vi "Test U8 Comm.vi"() -> ()   [LabVIEW 2021]
uses:
  ChannelCommon/typedef/Direction.ctl
  ChannelCommon/typedef/TimeStamps.ctl
  CIF_Iceoryx_PCAP_Universal.lvclass
  Iceorxy Utilities/Typedef/PCAP Config.ctl
  ChannelCommon/typedef/New FIFO Config.ctl
  ChannelCommon/typedef/FIFO Flags.ctl
  Iceorxy Utilities/Typedef/PCAP Linktype.ctl
  ChannelCommon/ChannelCommon.lvlib
  Iceorxy Utilities/Iceoryx Channel Utilities.lvlib
panel:
  out "status":string
  out "pass":bool
  out "error out":errorcluster
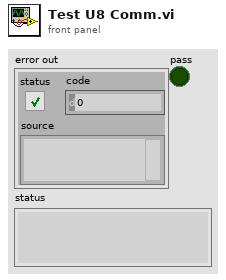
[diagram p1: front panel]
types:
  T1 = typedef "ChannelCommon.lvlib/Direction.ctl" = enum8{"Publisher", "Subscriber"}
  T2 = typedef "Iceoryx Channel Utilities.lvlib/PCAP Config.ctl" = cluster{"New FIFO Config":T3, "Linktype":T5, "Linktype Override":u32, "Type Name Override":string}
  T3 = typedef "ChannelCommon.lvlib/New FIFO Config.ctl" = cluster{"Max Bytes/Msg":u64, "Max Msg/FIFO":u64, "FIFO Flags":T4, "Best Effort Subscribers":u32, "Backpressure Subscribers":u32}
  T4 = typedef "ChannelCommon.lvlib/FIFO Flags.ctl" = cluster{"Backpressure":bool, "Extended Config":bool}
  T5 = typedef "Iceoryx Channel Utilities.lvlib/PCAP Linktype.ctl" = u32
  T6 = typedef "ChannelCommon.lvlib/TimeStamps.ctl" = cluster{"ClockID":u8, "T0":i64, "T_Out":i64}
  T7 = typedef "ChannelCommon.lvlib/New FIFO Instance Response.ctl" = cluster{"Publisher":string, "Custom Data":u8[]}
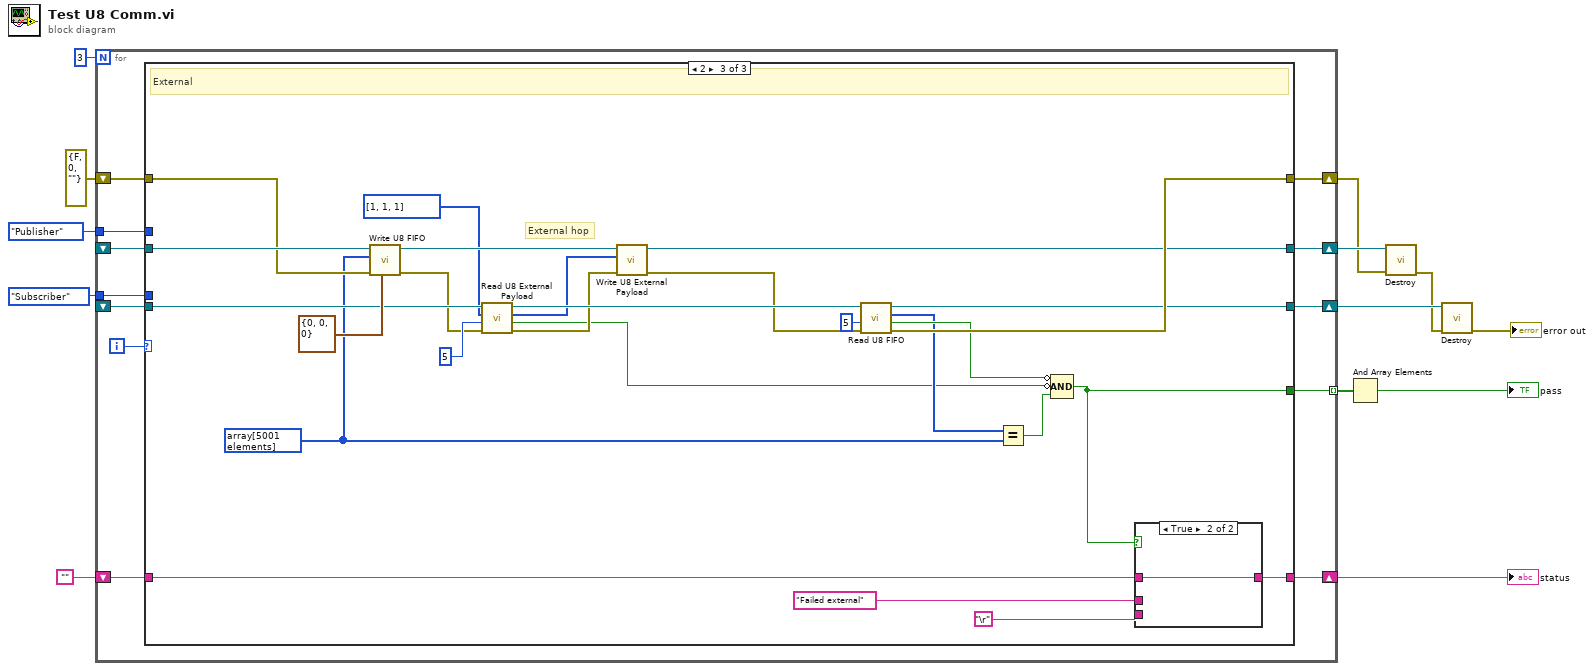
[diagram p0: block diagram]
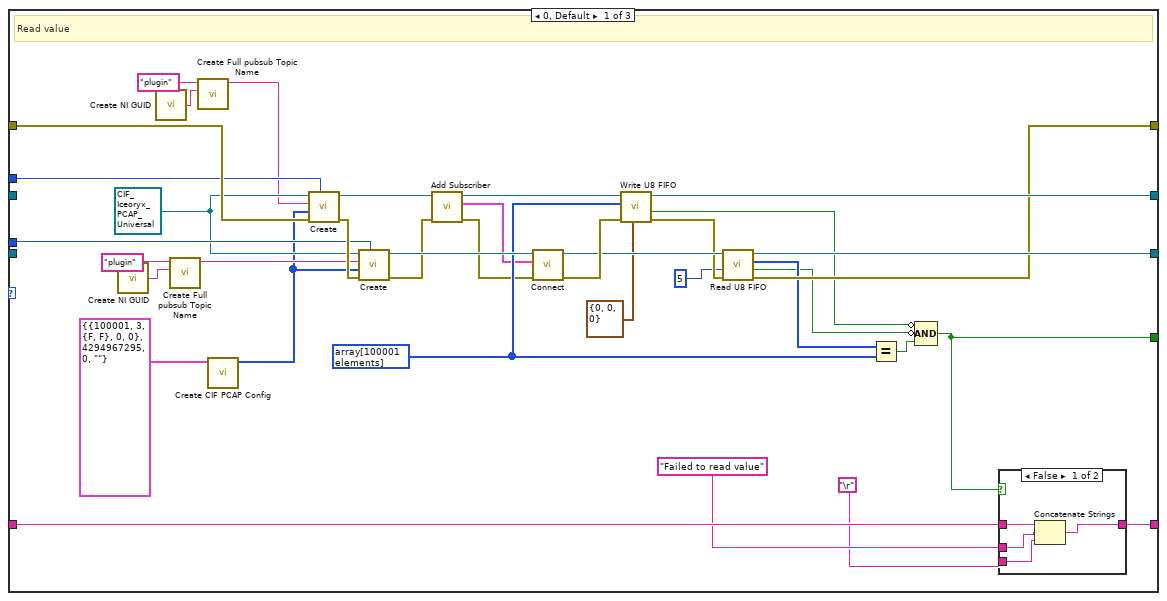
[diagram p2: hidden frame]
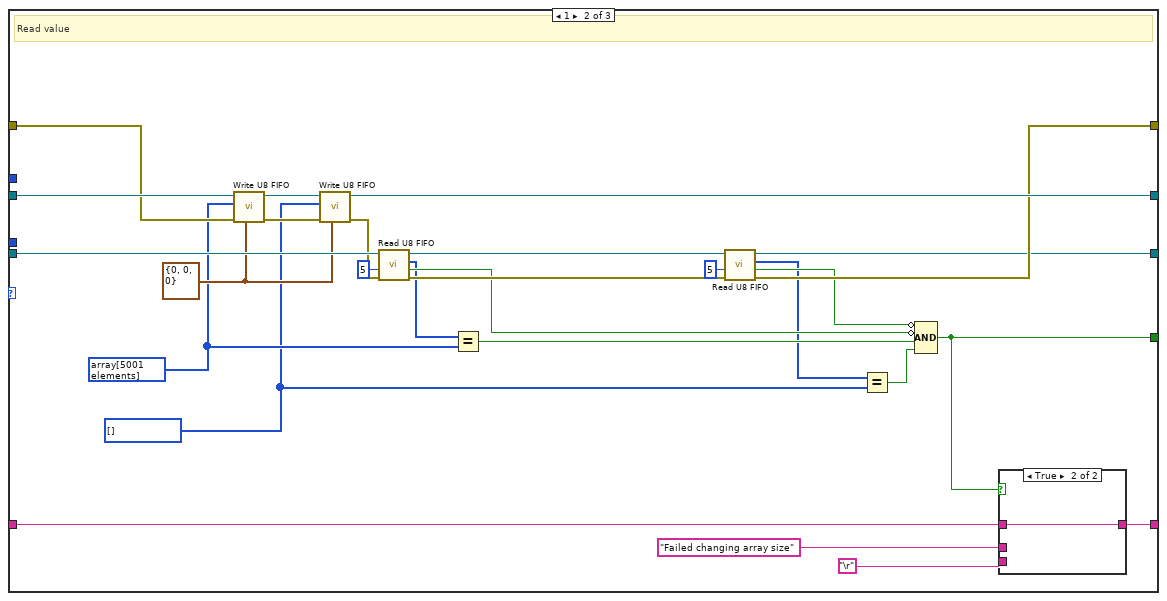
[diagram p4: hidden frame]
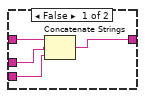
[diagram p5: hidden frame]
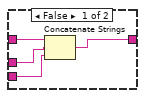
[diagram p6: hidden frame]
diagram:
  n1 = for {
    N: 3 -> [_]
    tunnel: [w25] -> w13 mode=indexing
    shift-right: [w23] -> w3
    shift-left: errorcluster {"status"=FALSE, "code"=0, "source"=""} ("error out") -> [w24]
    shift-right: [w20] -> w9
    shift-left: "" -> [w21]
    tunnel: Direction."Subscriber" ("Direction") -> [w19]
    tunnel: Direction."Publisher" ("Direction") -> [w18]
    shift-right: [w17] -> w5
    shift-left: _ -> [w15]
    shift-right: [w16] -> w4
    shift-left: _ -> [w14]
    i -> [w22]
    n2 = case shown="2" w22 {
      tunnel: [w57 w90 w121] -> w25
      tunnel: w24 -> [w55 w86 w118]
      tunnel: [w47 w79 w117] -> w23
      tunnel: w21 -> [w62 w94 w125]
      tunnel: [w61 w93 w124] -> w20
      tunnel: w19 -> [w54 _ _]
      tunnel: w18 -> [w53 _ _]
      tunnel: [w48 w76 w115] -> w17
      tunnel: [w50 w83 w103] -> w16
      tunnel: w14 -> [_ w87 w119]
      tunnel: w15 -> [_ w82 w111]
      frame 0, Default {
        w40 = refnum<class "CIF_Iceoryx_PCAP_Universal.lvclass"> refnum ("CIF_CIPC_Fifo_U8.lvclass")
        w41 = u8[] array[100001 elements] ("U8 Data")
        # "Read value"
        n3 = call <vilib>:"Create NI GUID.vi"() -> ("NI GUID"=w29:string)
        n4 = call <vilib>:"Create NI GUID.vi"() -> ("NI GUID"=w32:string)
        n5 = call "Create Full pubsub Topic Name.vi"("Topic"=w29, "Plugin name"="plugin") -> ("Full Topic"=w28:string)  [unwired: 8 in, 1 out]
        n6 = call "Create Full pubsub Topic Name.vi"("Topic"=w32, "Plugin name"="plugin") -> ("Full Topic"=w31:string)  [unwired: 8 in, 1 out]
        n7 = call "Create CIF PCAP Config.vi"("PCAP FIFO Config"=T2 {"New FIFO Config"={"Max Bytes/Msg"=100001, "Max Msg/FIFO"=3, "FIFO Flags"={"Backpressure"=FALSE, "Extended Config"=FALSE}, "Best Effort Subscribers"=0, "Backpressure Subscribers"=0}, "Linktype"=4294967295, "Linktype Override"=0, "Type Name Override"=""}) -> ("Flattened PCAP FIFO Config"=w26:u8[])  [unwired: 10 in]
        n8 = call-dynamic "Create.vi"("Direction"=w53, "error in (no error)"=w55, "Custom Config Data"=w26, "Name"=w31, "CIFFIFO in"=w40) -> ("error out"=w56:errorcluster, "CIFFIFO out"=w38:refnum<class "CIF_Iceoryx_PCAP_Universal.lvclass">)  [unwired: 5 in]
        n9 = call-dynamic "Create.vi"("Direction"=w54, "error in (no error)"=w56, "Custom Config Data"=w26, "Name"=w28, "CIFFIFO in"=w40) -> ("error out"=w35:errorcluster, "CIFFIFO out"=w52:refnum<class "CIF_Iceoryx_PCAP_Universal.lvclass">)  [unwired: 5 in]
        n10 = call-dynamic "Add Subscriber.vi"("error in (no error)"=w35, "CIF_CIPC_Chn in"=w38) -> ("error out"=w34:errorcluster, "New FIFO Instance"=w36:T7, "CIF_CIPC_Chn out"=w37:refnum<class "CIF_Iceoryx_PCAP_Universal.lvclass">)  [unwired: 7 in]
        n11 = call-dynamic "Connect.vi"("error in (no error)"=w34, "Connection"=w36, "CIF_Iceoryx_PCAP"=w52) -> ("error out"=w51:errorcluster, "CIF_Iceoryx_PCAP"=w49:refnum<class "CIF_Iceoryx_PCAP_Universal.lvclass">)  [unwired: 7 in]
        n12 = call-dynamic "Write U8 FIFO.vi"("FIFO Timestamps"=T6 {"ClockID"=0, "T0"=0, "T_Out"=0}, "error in (no error)"=w51, "Data in"=w41, "CIFFIFO in"=w37) -> ("error out"=w46:errorcluster, "timed out?"=w45:bool, "CIFFIFO out"=w50:refnum<class "CIF_Iceoryx_PCAP_Universal.lvclass">)  [unwired: 4 in, 1 out]
        n13 = call-dynamic "Read U8 FIFO.vi"("error in (no error)"=w46, "Timeout (ms)"=5, "CIFFIFO in"=w49) -> ("error out"=w47:errorcluster, "timed out?"=w43:bool, "Data out"=w44:u8[], "CIFFIFO out"=w48:refnum<class "CIF_Iceoryx_PCAP_Universal.lvclass">)  [unwired: 4 in, 1 out]
        n14 = Equal?(x=w44, y=w41) -> (x = y?=w58:bool)
        n15 = Compound Arithmetic op=AND(invert w45, invert w43, w58) -> (w57:bool)
        n16 = case shown="False" w57 {
          tunnel: w62 -> [w66 w67]
          tunnel: [w63 w67] -> w61
          tunnel: "Failed to read value" -> [w65 _]
          tunnel: "\r" -> [w64 _]
          frame False {
            n17 = Concatenate Strings(w66, w65, w64) -> (w63:string)
          }
          frame True {
          }
        }
      }
      frame 1 {
        w68 = u8[] [] ("U8 Data")
        w69 = u8[] array[5001 elements] ("U8 Data")
        w70 = T6 {"ClockID"=0, "T0"=0, "T_Out"=0} ("FIFO Timestamps")
        # "Read value"
        n18 = call-dynamic "Write U8 FIFO.vi"("FIFO Timestamps"=w70, "error in (no error)"=w86, "Data in"=w69, "CIFFIFO in"=w87) -> ("error out"=w84:errorcluster, "CIFFIFO out"=w85:refnum<class "CIF_Iceoryx_PCAP_Universal.lvclass">)  [unwired: 4 in, 2 out]
        n19 = call-dynamic "Write U8 FIFO.vi"("FIFO Timestamps"=w70, "error in (no error)"=w84, "Data in"=w68, "CIFFIFO in"=w85) -> ("error out"=w80:errorcluster, "CIFFIFO out"=w83:refnum<class "CIF_Iceoryx_PCAP_Universal.lvclass">)  [unwired: 4 in, 2 out]
        n20 = call-dynamic "Read U8 FIFO.vi"("error in (no error)"=w80, "Timeout (ms)"=5, "CIFFIFO in"=w82) -> ("error out"=w78:errorcluster, "timed out?"=w74:bool, "Data out"=w71:u8[], "CIFFIFO out"=w75:refnum<class "CIF_Iceoryx_PCAP_Universal.lvclass">)  [unwired: 4 in, 1 out]
        n21 = Equal?(x=w71, y=w69) -> (x = y?=w88:bool)
        n22 = call-dynamic "Read U8 FIFO.vi"("error in (no error)"=w78, "Timeout (ms)"=5, "CIFFIFO in"=w75) -> ("error out"=w79:errorcluster, "timed out?"=w73:bool, "Data out"=w72:u8[], "CIFFIFO out"=w76:refnum<class "CIF_Iceoryx_PCAP_Universal.lvclass">)  [unwired: 4 in, 1 out]
        n23 = Equal?(x=w72, y=w68) -> (x = y?=w89:bool)
        n24 = Compound Arithmetic op=AND(invert w73, invert w74, w88, w89) -> (w90:bool)
        n25 = case shown="True" w90 {
          tunnel: w94 -> [w98 w99]
          tunnel: [w95 w99] -> w93
          tunnel: "Failed changing array size" -> [w97 _]
          tunnel: "\r" -> [w96 _]
          frame False {
            n26 = Concatenate Strings(w98, w97, w96) -> (w95:string)
          }
          frame True {
          }
        }
      }
      frame 2 {
        w101 = u8[] array[5001 elements] ("U8 Data")
        # "External hop"
        # "External"
        n27 = call-dynamic "Write U8 FIFO.vi"("FIFO Timestamps"=T6 {"ClockID"=0, "T0"=0, "T_Out"=0}, "error in (no error)"=w118, "Data in"=w101, "CIFFIFO in"=w119) -> ("error out"=w104:errorcluster, "CIFFIFO out"=w105:refnum<class "CIF_Iceoryx_PCAP_Universal.lvclass">)  [unwired: 4 in, 2 out]
        n28 = call-dynamic "Read U8 External Payload.vi"("error in (no error)"=w104, "Timeout (ms)"=5, "Data in"=u8[] [1, 1, 1] ("U8 Data"), "CIF_Iceoryx_PCAP_Universal in"=w111) -> ("error out"=w109:errorcluster, "timed out?"=w107:bool, "Data out"=w108:u8[], "CIF_Iceoryx_PCAP_Universal out"=w110:refnum<class "CIF_Iceoryx_PCAP_Universal.lvclass">)  [unwired: 3 in, 1 out]
        n29 = call-dynamic "Write U8 External Payload.vi"("error in (no error)"=w109, "U8 With Header in"=w108, "CIF_Iceoryx_PCAP_Universal in"=w105) -> ("error out"=w102:errorcluster, "CIF_Iceoryx_PCAP_Universal out"=w103:refnum<class "CIF_Iceoryx_PCAP_Universal.lvclass">)  [unwired: 5 in, 2 out]
        n30 = call-dynamic "Read U8 FIFO.vi"("error in (no error)"=w102, "Timeout (ms)"=5, "CIFFIFO in"=w110) -> ("error out"=w117:errorcluster, "timed out?"=w114:bool, "Data out"=w113:u8[], "CIFFIFO out"=w115:refnum<class "CIF_Iceoryx_PCAP_Universal.lvclass">)  [unwired: 4 in, 1 out]
        n31 = Equal?(x=w113, y=w101) -> (x = y?=w120:bool)
        n32 = Compound Arithmetic op=AND(invert w114, invert w107, w120) -> (w121:bool)
        n33 = case shown="True" w121 {
          tunnel: w125 -> [w129 w130]
          tunnel: [w126 w130] -> w124
          tunnel: "Failed external" -> [w128 _]
          tunnel: "\r" -> [w127 _]
          frame False {
            n34 = Concatenate Strings(w129, w128, w127) -> (w126:string)
          }
          frame True {
          }
        }
      }
    }
  }
  "status" <- w9
  n35 = And Array Elements(Boolean array=w13) -> (logical AND=→"pass":bool)
  n36 = call-dynamic "Destroy.vi"("error in (no error)"=w3, "Icoryx_PCAP in"=w4) -> ("error out"=w2:errorcluster)  [unwired: 8 in, 1 out]
  n37 = call-dynamic "Destroy.vi"("error in (no error)"=w2, "Icoryx_PCAP in"=w5) -> ("error out"=→"error out":errorcluster)  [unwired: 8 in, 1 out]
